vi "SeqEditor_DATALOAD.vi"(8 "error in (no error)":errorcluster, 11 "NLTest in":refnum<class "NLTest.lvclass">) -> (0 "error out":errorcluster, 3 "NLTest out":refnum<class "NLTest.lvclass">)   [LabVIEW 2017, in "NLTest.lvclass"]
uses:
  NLTest.lvclass
  allseqanddata.ctl
  NLTest.lvclass/NLTest.ctl
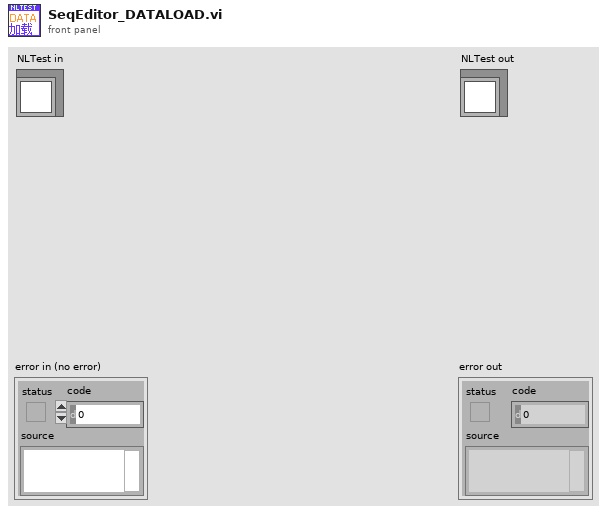
[diagram p1: front panel]
types:
  T1 = typedef "NLTest.lvclass/allseqanddata.ctl" = cluster{"seqname":string, "seqdata":string[]}
  T2 = enum16{"open", "replace", "create", "open or create", "replace or create", "replace or create with confirmation"}
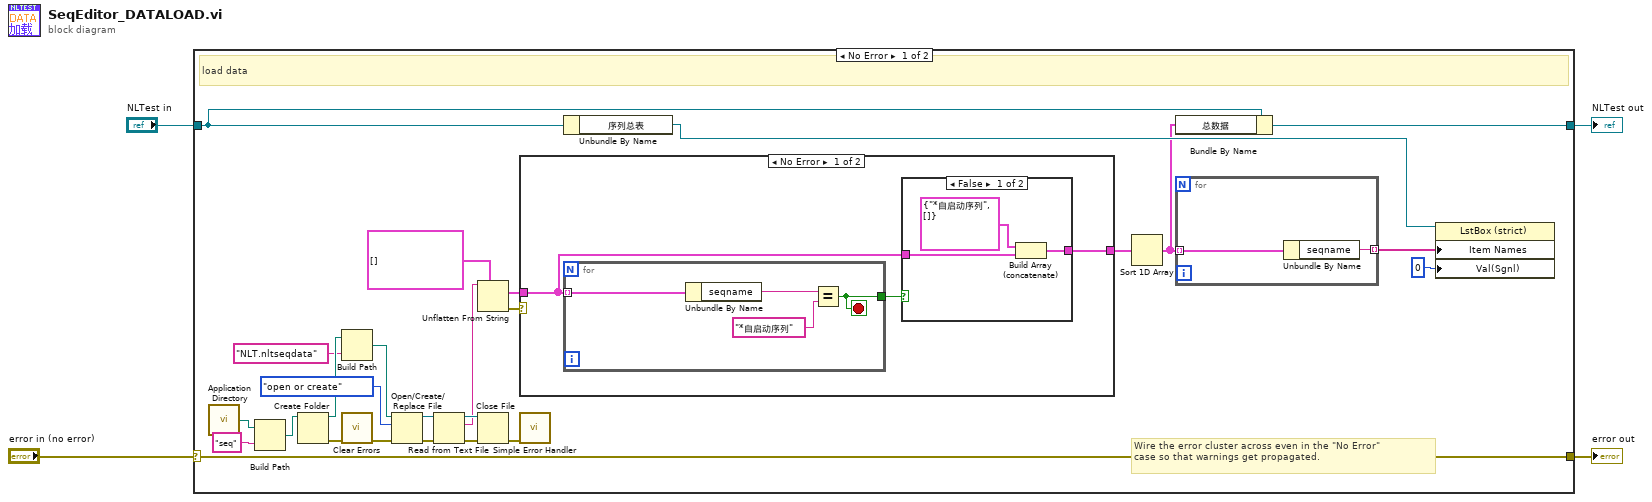
[diagram p0: block diagram]
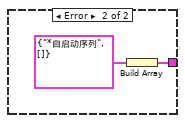
[diagram p3: hidden frame]
diagram:
  n1 = case shown="No Error" "error in (no error)" {
    selector: "error in (no error)" -> [w30 w47]
    tunnel: [w30 w47] -> w3
    tunnel: [w10 w46] -> w1
    tunnel: "NLTest in" -> [w11 w46]
    frame No Error {
      # "Wire the error cluster across even in the \"No Error\"\ncase so that warnings get propagated."
      # "load data"
      n2 = call <vilib>:"Application Directory.vi"() -> ("Application Directory"=w29:path)
      n3 = Build Path(base path=w29, name or relative path="seq") -> (appended path=w28:path)
      n4 = Create Folder(path (use dialog)=w28) -> (created path=w24:path, error out=w26:errorcluster)  [unwired: 2 in, 1 out]
      n5 = Build Path(base path=w24, name or relative path="NLT.nltseqdata") -> (appended path=w22:path)
      n6 = call <vilib>:"Clear Errors.vi"("error in (no error)"=w26) -> ("error out"=w25:errorcluster)  [unwired: 5 in, 1 out]
      n7 = Open/Create/Replace File(file path (use dialog)=w22, error in=w25, operation (0:open)=T2."open or create") -> (refnum out=w19:refnum<file>, error out=w20:errorcluster)  [unwired: 3 in, 1 out]
      n8 = Read from Text File(file (use dialog)=w19, error in=w20) -> (refnum out=w17:refnum<file>, text=w15:string, error out=w18:errorcluster)  [unwired: 2 in, 1 out]
      n9 = Unflatten From String(type=T1[] [] ("Array"), binary string=w15) -> (value=w12:T1[], error out=w13:errorcluster)  [unwired: 3 in, 1 out]
      n10 = Close File(refnum=w17, error in=w18) -> (error out=w16:errorcluster)  [unwired: 1 out]
      n11 = case shown="No Error" w13 {
        tunnel: w12 -> [w33 _]
        tunnel: [w34 w44] -> w6
        frame No Error {
          n12 = for {
            tunnel: w33 -> [w43] mode=indexing
            tunnel: [w40] -> w35
            stop <- w40 stop-if-true
            n13 = Unbundle By Name(w43) -> ("seqname"=w42:string)
            n14 = Equal?(x=w42, y="*自启动序列" ("element")) -> (x = y?=w40:bool)
          }
          n15 = case shown="False" w35 {
            tunnel: [w36 w39] -> w34
            tunnel: w33 -> [w37 w39]
            frame False {
              n16 = Build Array (concatenate)(T1 {"seqname"="*自启动序列", "seqdata"=[]} ("allseqanddata"), w37) -> (w36:T1[])
            }
            frame True {
            }
          }
        }
        frame Error {
          n17 = Build Array(T1 {"seqname"="*自启动序列", "seqdata"=[]} ("allseqanddata")) -> (w44:T1[])
        }
      }
      n18 = call <vilib>:"Simple Error Handler.vi"("error in (no error)"=w16) -> ()  [unwired: 4 in, 5 out]
      n19 = Unbundle By Name(w11) -> ("序列总表"=w9:refnum<vi>)
      n20 = Sort 1D Array(array=w6) -> (sorted array=w5:T1[])
      n21 = Bundle By Name(cluster=w11, "总数据"=w5) -> (w10:refnum<class "NLTest.lvclass">)
      n22 = for {
        tunnel: w5 -> [w32] mode=indexing
        tunnel: [w31] -> w8 mode=indexing
        n23 = Unbundle By Name(w32) -> ("seqname"=w31:string)
      }
      n24 = property class="LstBox (strict)"(reference=w9, "Item Names"=w8, "Val(Sgnl)"=0 ("Value (Signaling)")) -> ()  [unwired: 1 in, 2 out]
    }
    frame Error {
    }
  }
  "error out" <- w3
  "NLTest out" <- w1
